vi "SUP_Camera_FrameTap.vi"(5 "error in (no error)":errorcluster, 6 "Image":T1, 7 "valeur de l'horloge en ms 3":u32, 8 "SetupOK":bool, 9 "valeur de l'horloge en ms 2":u32, 10 "temps actuel":timestamp, 11 "valeur de l'horloge en ms":u32) -> (0 "valid_for_run":bool, 1 "channel_out":u32, 2 "capture":timestamp, 3 "error in (no error) 2":errorcluster, 4 "Image 2":T1)   [LabVIEW 2012]
uses:
  <vilib>/vision/Image Controls.llb/IMAQ Image.ctl
panel:
  in  "temps actuel 3":timestamp
  out "error in (no error) 3":errorcluster
  in  "temps actuel 2":timestamp
  out "Image Pixels (I16)":i16[][](array[numeric])
  out "Image Pixels (U8)":u8[][](array[numeric])
  out "error out":errorcluster
  out "Image Pixels (Float)":sgl[][](array[numeric]) format="%.2f"
  out "Image Pixels (U16)":u16[][](array[numeric])
  in  "Optional Rectangle":i32[](array[numeric])
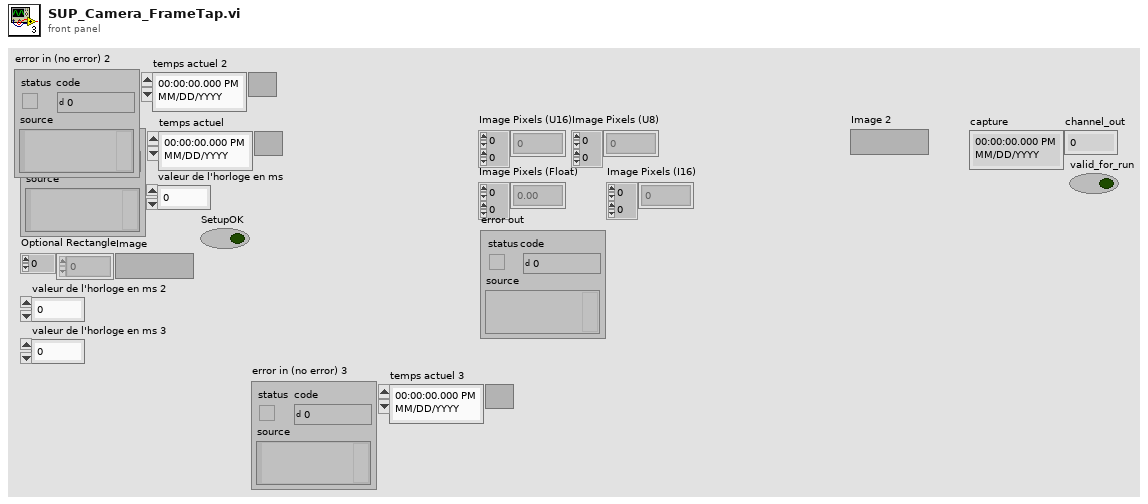
[diagram p1: front panel]
types:
  T1 = typedef "IMAQ Image.ctl" = refnum<image>
  T2 = cluster{"temps actuel":timestamp, "capture":timestamp, "millisecond timer value":u32, "valeur de l'horloge en ms 3":u32, bool, bool}
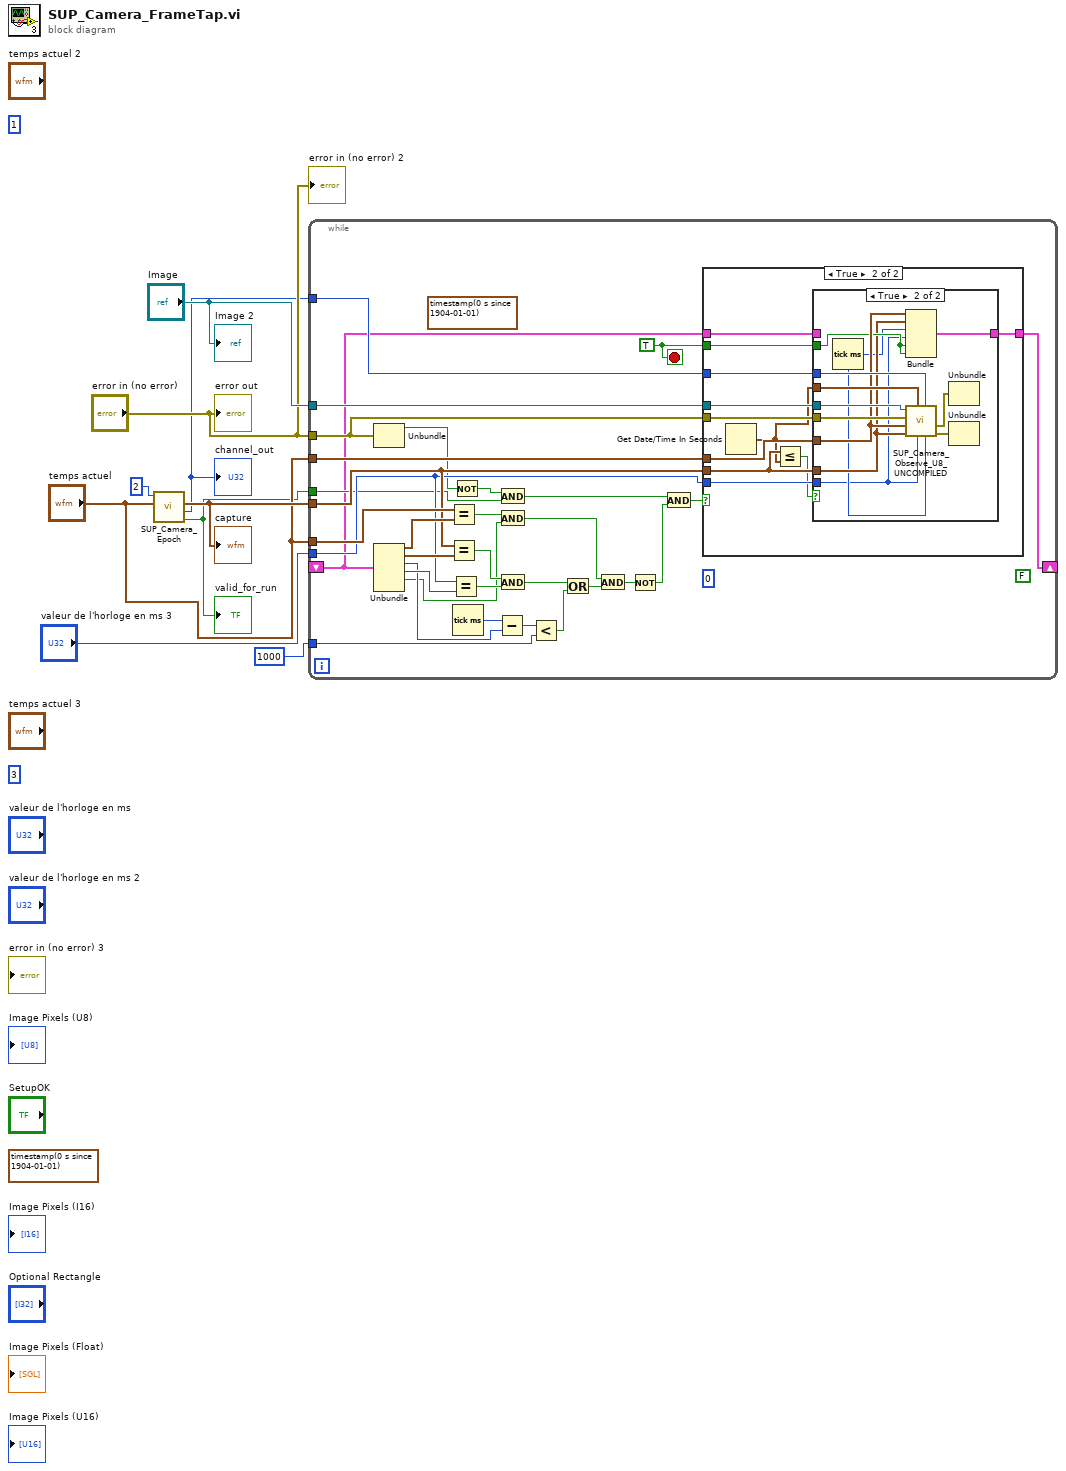
[diagram p0: block diagram]
diagram:
  (unwired) u32 3 ("valeur de l'horloge en ms 2")
  (unwired) u32 1 ("valeur de l'horloge en ms 2")
  (unwired) timestamp(0 s since 1904-01-01) ("temps actuel 3")
  n1 = call "SUP_Camera_Epoch.vi"("temps actuel"="temps actuel", "valeur de l'horloge en ms"=u32 2 ("valeur de l'horloge en ms 2")) -> ("valid_for_run"=w1:bool, "channel_out"=w2:u32, "capture"=w6:timestamp)  [unwired: 5 in, 2 out]
  "capture" <- w6
  "channel_out" <- w2
  "valid_for_run" <- w1
  n2 = while {
    shift-right: [w11] -> _
    shift-left: _ -> [w10]
    tunnel: "Image" -> [w41]
    tunnel: "error in (no error)" -> [w19]
    tunnel: "temps actuel" -> [w40]
    tunnel: w6 -> [w36]
    tunnel: "valeur de l'horloge en ms 3" -> [w34]
    tunnel: w2 -> [w39]
    tunnel: "temps actuel" -> [w38]
    tunnel: u32 1000 ("valeur de l'horloge en ms 2") -> [w29]
    tunnel: w1 -> [w16]
    stop <- w12 stop-if-true
    (unwired) FALSE ("SetupOK")
    (unwired) u32 0 ("valeur de l'horloge en ms 2")
    w12 = TRUE
    (unwired) timestamp(0 s since 1904-01-01) ("temps actuel 3")
    n3 = Unbundle(w19) -> ("status"=w18:bool)  [unwired: 2 out]
    n4 = Unbundle(w10) -> ("temps actuel"=w37:timestamp, "capture"=w35:timestamp, "millisecond timer value"=w31:u32, "valeur de l'horloge en ms 3"=w33:u32, w23:bool)  [unwired: 1 out]
    n5 = Equal?(x=w38, y=w37) -> (x = y?=w24:bool)
    n6 = Equal?(x=w36, y=w35) -> (x = y?=w28:bool)
    n7 = Equal?(x=w34, y=w33) -> (x = y?=w27:bool)
    n8 = Not(x=w18) -> (.not. x?=w17:bool)
    n9 = Tick Count (ms)() -> (millisecond timer value=w32:u32)
    n10 = Subtract(x=w32, y=w31) -> (x-y=w30:u32)
    n11 = And(x=w17, y=w16) -> (x .and. y?=w15:bool)
    n12 = And(x=w24, y=w23) -> (x .and. y?=w22:bool)
    n13 = And(x=w28, y=w27) -> (x .and. y?=w26:bool)
    n14 = Less?(x=w30, y=w29) -> (x < y?=w25:bool)
    n15 = Or(x=w26, y=w25) -> (x .or. y?=w21:bool)
    n16 = And(x=w22, y=w21) -> (x .and. y?=w20:bool)
    n17 = Not(x=w20) -> (.not. x?=w14:bool)
    n18 = And(x=w15, y=w14) -> (x .and. y?=w13:bool)
    n19 = case shown="True" w13 {
      tunnel: w41 -> [_ w53]
      tunnel: w19 -> [_ w52]
      tunnel: w40 -> [_ w51]
      tunnel: w36 -> [_ w48]
      tunnel: w34 -> [_ w50]
      tunnel: w39 -> [_ w49]
      tunnel: w12 -> [_ w45]
      tunnel: [w42 w44] -> w11
      tunnel: w10 -> [w42 w43]
      frame False {
      }
      frame True {
        n20 = Get Date/Time In Seconds() -> (seconds since 1Jan1904=w46:timestamp)
        n21 = Less Or Equal?(x=w48, y=w46) -> (x <= y?=w47:bool)
        n22 = case shown="True" w47 {
          tunnel: w53 -> [_ w66]
          tunnel: w52 -> [_ w65]
          tunnel: w51 -> [_ w60]
          tunnel: w50 -> [_ w55]
          tunnel: w49 -> [_ w64]
          tunnel: w48 -> [_ w57]
          tunnel: w46 -> [_ w61]
          tunnel: w45 -> [_ w59]
          tunnel: [w54 w58] -> w44
          tunnel: w43 -> [w54 _]
          frame False {
          }
          frame True {
            n23 = Tick Count (ms)() -> (millisecond timer value=w56:u32)
            n24 = Bundle("temps actuel"=w60, "capture"=w57, "millisecond timer value"=w56, "valeur de l'horloge en ms 3"=w55, w59, w59) -> (w58:T2)  [unwired: 1 in]
            n25 = call "SUP_Camera_Observe_U8_UNCOMPILED.vi"("valeur de l'horloge en ms 3"=w56, "valeur de l'horloge en ms 2"=w64, "valeur de l'horloge en ms"=w55, "temps actuel 3"=w61, "temps actuel 2"=w57, "temps actuel"=w60, "error in (no error)"=w65, "Image"=w66) -> ("error out"=w62:errorcluster, "error in (no error) 3"=w63:errorcluster)  [unwired: 2 out]
            n26 = Unbundle(w63) -> ()  [unwired: 3 out]
            n27 = Unbundle(w62) -> ()  [unwired: 3 out]
          }
        }
      }
    }
  }
  "error out" <- "error in (no error)"
  "error in (no error) 2" <- "error in (no error)"
  "Image 2" <- "Image"
